vi "FiSens UDP example program_LV2014.vi"() -> ()   [LabVIEW 2014]
panel:
  in  "Zero Spectrometer":bool
  out "time (s)":dbl format="%.3f"
  out "Sensor array":T1(array[cluster]) {"Strain (µm/m)" format="%.2f"; "Temperature (°C)" format="%.2f"; "WL FBG (nm)" format="%.4g"; "WL Temp FBG (nm)" format="%.4f"; "Amp FBG" format="%#.3f"; "Amp Temp FBG" format="%.2f"}
  in  "Masterstop":bool
  in  "UDP Settings to BraggSens":T2={"BragSens UDP Port"=16000, "example program UDP-Port"=16001, "BraggSens IP address"="localhost", "example program IP-Addresse"="localhost"}
  out "received String":string
  in  "Connect Spectrometer":bool
  out "Listening on UDP":bool
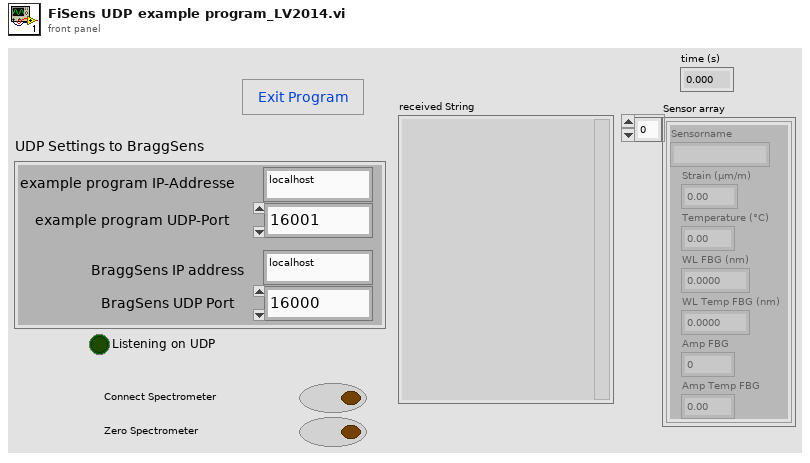
[diagram p1: front panel]
types:
  T1 = cluster{"Sensorname":string, "Strain (µm/m)":dbl, "Temperature (°C)":dbl, "WL FBG (nm)":dbl, "WL Temp FBG (nm)":dbl, "Amp FBG":dbl, "Amp Temp FBG":dbl}[]
  T2 = cluster{"BragSens UDP Port":i32, "example program UDP-Port":i32, "BraggSens IP address":string, "example program IP-Addresse":string}
  T3 = cluster{"Sensorname":string, "Strain (µm/m)":dbl, "Temperature (°C)":dbl, "WL FBG (nm)":dbl, "WL Temp FBG (nm)":dbl, "Amp FBG":dbl, "Amp Temp FBG":dbl}
  T4 = cluster{"BragSens UDP Port":bool, "example program UDP-Port":bool, "BraggSens IP address":bool, "example program IP-Addresse":bool}
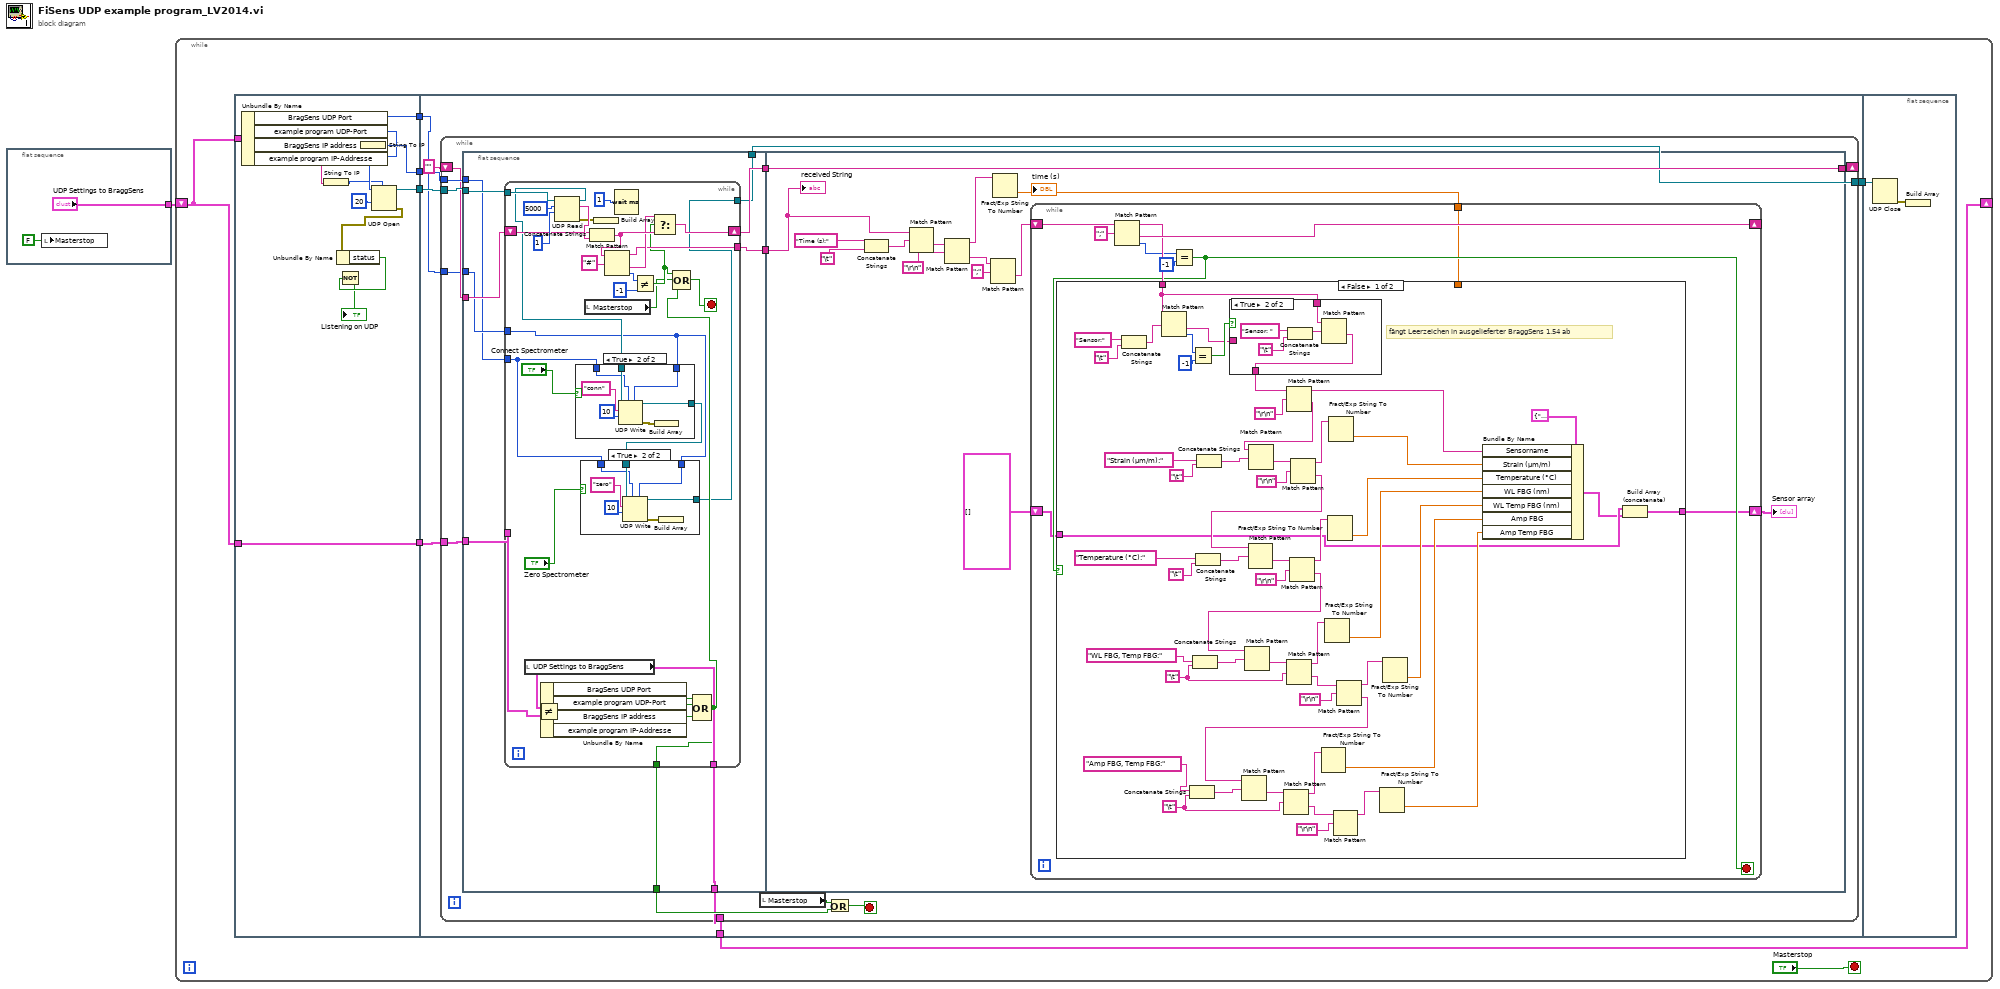
[diagram p0: block diagram]
diagram:
  n1 = flat-sequence {
    tunnel: ["UDP Settings to BraggSens"] -> w1
    frame #0 {
      n2 = local write "Masterstop"(FALSE ("Masterstop")) -> ()
    }
  }
  n3 = while {
    shift-right: [w5] -> _
    shift-left: w1 -> [w6]
    stop <- "Masterstop" stop-if-true
    n4 = flat-sequence {
      tunnel: [w23] -> w11
      tunnel: [w21] -> w10
      tunnel: [w20] -> w9
      tunnel: w6 -> [w16]
      tunnel: w6 -> [w15]
      tunnel: [w15] -> w7
      tunnel: w11 -> [w30]
      tunnel: w10 -> [w31]
      tunnel: w9 -> [w28]
      tunnel: [w27] -> w8
      tunnel: w7 -> [w26]
      tunnel: [w25] -> w5
      tunnel: w8 -> [w188]
      frame #0 {
        n5 = Unbundle By Name(w16) -> ("BragSens UDP Port"=w20:i32, "example program UDP-Port"=w19:i32, "BraggSens IP address"=w22:string, "example program IP-Addresse"=w18:string)
        n6 = String To IP(1:w18) -> (0:w17:u32)
        n7 = String To IP(1:w22) -> (0:w21:u32)
        n8 = UDP Open(7:w17, 9:20, 11:w19) -> (port=w23:refnum<k16>, 0:w14:errorcluster)  [unwired: 2 in, 1 out]
        n9 = Unbundle By Name(w14) -> ("status"=w13:bool)
        n10 = Not(x=w13) -> (.not. x?=→"Listening on UDP":bool)
      }
      frame #1 {
        n11 = while {
          tunnel: w30 -> [w44]
          tunnel: w31 -> [w43]
          shift-right: [w38] -> _
          shift-left: "" -> [w42]
          tunnel: w28 -> [w41]
          tunnel: [w37] -> w27
          tunnel: w26 -> [w34]
          tunnel: [w32] -> w25
          stop <- w35 stop-if-true
          n12 = flat-sequence {
            tunnel: w44 -> [w54]
            tunnel: w43 -> [w51]
            tunnel: w42 -> [w53]
            tunnel: w41 -> [w52]
            tunnel: [w50] -> w40
            tunnel: [w49] -> w39
            tunnel: [w48] -> w37
            tunnel: w34 -> [w47]
            tunnel: [w46] -> w33
            tunnel: [w45] -> w32
            tunnel: w40 -> [w116]
            tunnel: w39 -> [w103]
            tunnel: [w116] -> w38
            frame #0 {
              n13 = while {
                shift-right: [w78] -> w50
                shift-left: w53 -> [w83]
                tunnel: [w76] -> w49
                tunnel: w54 -> [w74]
                tunnel: [w57] -> w48
                tunnel: w52 -> [w56]
                tunnel: w51 -> [w60]
                tunnel: w47 -> [w62]
                tunnel: [w61] -> w46
                tunnel: [w63] -> w45
                stop <- w70 stop-if-true
                n14 = local read "UDP Settings to BraggSens"() -> (w63:T2)
                n15 = Not Equal?(x=w63, y=w62) -> (x != y?=w68:T4)
                n16 = Unbundle By Name(w68) -> ("BragSens UDP Port"=w67:bool, "example program UDP-Port"=w66:bool, "BraggSens IP address"=w65:bool, "example program IP-Addresse"=w64:bool)
                n17 = UDP Read(connection ID=w74, max size (548)=5000, timeout ms (25000)=1 ("Timeout in ms (25000)")) -> (data out=w84:string, error out=w69:errorcluster, 3:w59:refnum<k16>)  [unwired: 1 in, 2 out]
                n18 = case shown="True" "Connect Spectrometer" {
                  tunnel: w59 -> [w95 w100]
                  tunnel: [w95 w99] -> w58
                  tunnel: w56 -> [_ w98]
                  tunnel: w60 -> [_ w97]
                  frame False {
                  }
                  frame True {
                    n19 = UDP Write ("UDP: Schreiben")(address=w97, port or service name=w98, connection ID=w100, data in="conn" ("Regulärer Ausdruck"), 9:10) -> (error out=w96:errorcluster, 3:w99:refnum<k16>)  [unwired: 1 in]
                    n20 = Build Array(w96) -> ()  [unwired: 1 out]
                  }
                }
                n21 = case shown="True" "Zero Spectrometer" {
                  tunnel: w58 -> [w87 w92]
                  tunnel: [w87 w91] -> w57
                  tunnel: w56 -> [_ w90]
                  tunnel: w60 -> [_ w89]
                  frame False {
                  }
                  frame True {
                    n22 = UDP Write ("UDP: Schreiben")(address=w89, port or service name=w90, connection ID=w92, data in="zero" ("Regulärer Ausdruck"), 9:10) -> (error out=w88:errorcluster, 3:w91:refnum<k16>)  [unwired: 1 in]
                    n23 = Build Array(w88) -> ()  [unwired: 1 out]
                  }
                }
                n24 = local read "Masterstop"() -> (w71:bool)
                n25 = Concatenate Strings(w83, w84) -> (w79:string)
                n26 = Build Array(w69) -> ()  [unwired: 1 out]
                n27 = Match Pattern(string=w79, regular expression="#" ("Regulärer Ausdruck")) -> (before substring=w76:string, after substring=w77:string, offset past match=w81:i32)  [unwired: 1 in, 1 out]
                n28 = Wait (ms)(milliseconds to wait=u32 1 ("Zu wartende ms")) -> ()  [unwired: 1 out]
                n29 = Not Equal?(x=w81, y=-1) -> (x != y?=w72:bool)
                n30 = Select(t=w77, s=w72, f=w79) -> (s? t:f=w78:string)
                n31 = Compound Arithmetic op=OR ("Mehrfacharithmetik")(w67, w66, w65, w64) -> (w61:bool)
                n32 = Compound Arithmetic op=OR ("Mehrfacharithmetik")(w72, w71, w61) -> (w70:bool)
              }
            }
            frame #1 {
              n33 = Concatenate Strings("Time (s):" ("Regulärer Ausdruck"), "\t") -> (w109:string)
              n34 = Match Pattern(string=w103, regular expression=w109) -> (after substring=w110:string)  [unwired: 1 in, 3 out]
              n35 = Match Pattern(string=w110, regular expression="\r\n") -> (before substring=w111:string, after substring=w112:string)  [unwired: 1 in, 2 out]
              n36 = Match Pattern(string=w112, regular expression=";" ("Regulärer Ausdruck")) -> (after substring=w113:string)  [unwired: 1 in, 3 out]
              n37 = Fract/Exp String To Number(string=w111) -> (number=w114:dbl)  [unwired: 3 in, 1 out]
              "time (s)" <- w114
              n38 = while {
                shift-right: [w124] -> _
                shift-left: w113 -> [w126]
                tunnel: w114 -> [w119]
                shift-right: [w118] -> w115
                shift-left: T1 [] -> [w117]
                stop <- w120 stop-if-true
                n39 = Match Pattern(string=w126, regular expression=";" ("Regulärer Ausdruck")) -> (before substring=w123:string, after substring=w124:string, offset past match=w122:i32)  [unwired: 1 in, 1 out]
                n40 = Equal?(x=w122, y=-1) -> (x = y?=w120:bool)
                n41 = case shown="False" w120 {
                  tunnel: w123 -> [w130 _]
                  tunnel: w119 -> [_ _]
                  tunnel: [w136 w186] -> w118
                  tunnel: w117 -> [w135 w186]
                  frame False {
                    w149 = "\t"
                    w156 = "\t"
                    # "fängt Leerzeichen in ausgelieferter BraggSens 1.54 ab"
                    n42 = Concatenate Strings("Sensor:", "\t") -> (w179:string)
                    n43 = Match Pattern(string=w130, regular expression=w179) -> (after substring=w129:string, offset past match=w132:i32)  [unwired: 1 in, 2 out]
                    n44 = Concatenate Strings("Amp FBG, Temp FBG:", w149) -> (w146:string)
                    n45 = Equal?(x=w132, y=-1) -> (x = y?=w131:bool)
                    n46 = Concatenate Strings("WL FBG, Temp FBG:", w156) -> (w161:string)
                    n47 = Concatenate Strings("Temperature (°C):", "\t") -> (w166:string)
                    n48 = Concatenate Strings("Strain (µm/m):", "\t") -> (w174:string)
                    n49 = case shown="True" w131 {
                      tunnel: w130 -> [_ w182]
                      tunnel: w129 -> [w180 _]
                      tunnel: [w180 w181] -> w128
                      frame False {
                      }
                      frame True {
                        n50 = Concatenate Strings("Sensor: ", "\t") -> (w183:string)
                        n51 = Match Pattern(string=w182, regular expression=w183) -> (after substring=w181:string)  [unwired: 1 in, 3 out]
                      }
                    }
                    n52 = Match Pattern(string=w128, regular expression="\r\n") -> (before substring=w143:string, after substring=w173:string)  [unwired: 1 in, 2 out]
                    n53 = Match Pattern(string=w173, regular expression=w174) -> (after substring=w171:string)  [unwired: 1 in, 3 out]
                    n54 = Match Pattern(string=w171, regular expression="\r\n") -> (before substring=w169:string, after substring=w164:string)  [unwired: 1 in, 2 out]
                    n55 = Match Pattern(string=w164, regular expression=w166) -> (after substring=w167:string)  [unwired: 1 in, 3 out]
                    n56 = Match Pattern(string=w167, regular expression="\r\n") -> (before substring=w162:string, after substring=w159:string)  [unwired: 1 in, 2 out]
                    n57 = Match Pattern(string=w159, regular expression=w161) -> (after substring=w160:string)  [unwired: 1 in, 3 out]
                    n58 = Match Pattern(string=w160, regular expression=w156) -> (before substring=w157:string, after substring=w154:string)  [unwired: 1 in, 2 out]
                    n59 = Fract/Exp String To Number(string=w157) -> (number=w140:dbl)  [unwired: 3 in, 1 out]
                    n60 = Fract/Exp String To Number(string=w162) -> (number=w141:dbl)  [unwired: 3 in, 1 out]
                    n61 = Fract/Exp String To Number(string=w169) -> (number=w142:dbl)  [unwired: 3 in, 1 out]
                    n62 = Match Pattern(string=w154, regular expression="\r\n") -> (before substring=w155:string, after substring=w145:string)  [unwired: 1 in, 2 out]
                    n63 = Match Pattern(string=w145, regular expression=w146) -> (after substring=w147:string)  [unwired: 1 in, 3 out]
                    n64 = Match Pattern(string=w147, regular expression=w149) -> (before substring=w148:string, after substring=w151:string)  [unwired: 1 in, 2 out]
                    n65 = Fract/Exp String To Number(string=w148) -> (number=w138:dbl)  [unwired: 3 in, 1 out]
                    n66 = Match Pattern(string=w151, regular expression="\r\n") -> (before substring=w150:string)  [unwired: 1 in, 3 out]
                    n67 = Fract/Exp String To Number(string=w150) -> (number=w137:dbl)  [unwired: 3 in, 1 out]
                    n68 = Fract/Exp String To Number(string=w155) -> (number=w139:dbl)  [unwired: 3 in, 1 out]
                    n69 = Bundle By Name(cluster=T3 {"Sensorname"="", "Strain (µm/m)"=0.0, "Temperature (°C)"=0.0, "WL FBG (nm)"=0.0, "WL Temp FBG (nm)"=0.0, "Amp FBG"=0.0, "Amp Temp FBG"=0.0} ("Ausgangs-Cluster"), "Sensorname"=w143, "Strain (µm/m)"=w142, "Temperature (°C)"=w141, "WL FBG (nm)"=w140, "WL Temp FBG (nm)"=w139, "Amp FBG"=w138, "Amp Temp FBG"=w137) -> (w134:T3)
                    n70 = Build Array (concatenate)(w135, w134) -> (w136:T1)
                  }
                  frame True {
                  }
                }
              }
              "Sensor array" <- w115
              "received String" <- w103
            }
          }
          n71 = local read "Masterstop"() -> (w36:bool)
          n72 = Or(x=w36, y=w33) -> (x .or. y?=w35:bool)
        }
      }
      frame #2 {
        n73 = UDP Close(connection ID=w188) -> (error out=w187:errorcluster)  [unwired: 1 in, 1 out]
        n74 = Build Array(w187) -> ()  [unwired: 1 out]
      }
    }
  }
